vi "Node Type.vi"(8 "error in (no error)":errorcluster, 11 "JSON Tree In":variant) -> (0 "error out":errorcluster, 2 "Value":variant, 3 "JSON Tree Out":variant, 5 "JSON Compatible Type":T1=enum."Unknown", 7 "JSON Type":T2=enum."Unknown")   [LabVIEW 2014, in "i3-json.lvlib"]
doc: "Returns the JSON Type and Value of a given node in a JSON Tree. If possible, will also tell if there is a compatible LabVIEW datatype."
uses:
  i3-json.lvlib
  JSON Types/JSON Type.ctl
  JSON Types/JSON Compatible Type.ctl
  JSON Types/JSON Variant Attribute.ctl
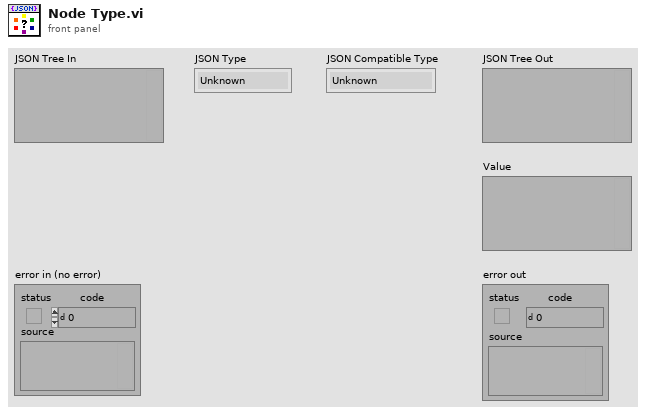
[diagram p1: front panel]
types:
  T1 = typedef "i3-json.lvlib/JSON Compatible Type.ctl" = enum16{"1D Double Array", "1D String Array", "1D Boolean Array", "Unknown"}
  T2 = typedef "i3-json.lvlib/JSON Type.ctl" = enum8{"JSON Compatible", "JSON Array", "JSON Object", "JSON Null", "Double", "String", "Boolean", "Unknown"}
  T3 = typedef "i3-json.lvlib/JSON Variant Attribute.ctl" = string
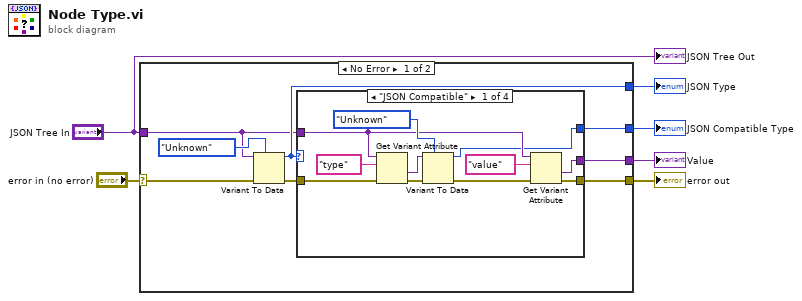
[diagram p0: block diagram]
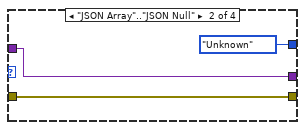
[diagram p2: hidden frame]
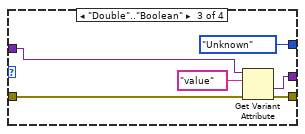
[diagram p3: hidden frame]
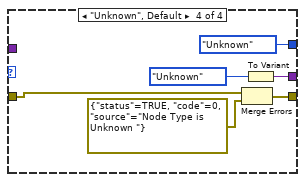
[diagram p4: hidden frame]
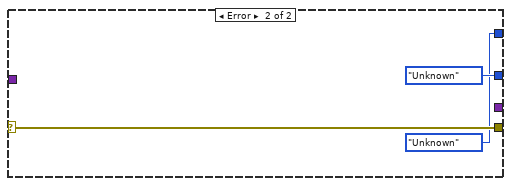
[diagram p5: hidden frame]
diagram:
  n1 = case shown="No Error" "error in (no error)" {
    selector: "error in (no error)" -> [w13 w43]
    tunnel: [w9 w43] -> w5
    tunnel: [w11 JSON_Compatible_Type."Unknown" ("JSON Compatible Type")] -> w4
    tunnel: [w10 JSON_Type."Unknown" ("JSON Type")] -> w3
    tunnel: "JSON Tree In" -> [w8 _]
    tunnel: [w7 _] -> w1
    frame No Error {
      n2 = Variant To Data(error in=w13, type=JSON_Type."Unknown" ("JSON Type"), Variant=w8) -> (data=w10:T2, error out=w12:errorcluster)
      n3 = case shown="\"JSON Compatible\"" w10 {
        tunnel: w8 -> [w17 w26 w33 _]
        tunnel: w12 -> [w25 w27 w31 w37]
        tunnel: [w15 JSON_Compatible_Type."Unknown" ("JSON Compatible Type") JSON_Compatible_Type."Unknown" ("JSON Compatible Type") JSON_Compatible_Type."Unknown" ("JSON Compatible Type")] -> w11
        tunnel: [w19 w27 w30 w35] -> w9
        tunnel: [w16 w26 w29 w40] -> w7
        frame "JSON Compatible" {
          n4 = Get Variant Attribute(Variant=w17, name=T3 "type" ("JSON Variant Attribute"), error in=w25) -> (value=w22:variant, error out=w23:errorcluster)  [unwired: 1 in, 2 out]
          n5 = Variant To Data(error in=w23, type=JSON_Compatible_Type."Unknown" ("JSON Compatible Type"), Variant=w22) -> (data=w15:T1, error out=w20:errorcluster)
          n6 = Get Variant Attribute(Variant=w17, name=T3 "value" ("JSON Variant Attribute"), error in=w20) -> (value=w16:variant, error out=w19:errorcluster)  [unwired: 1 in, 2 out]
        }
        frame "JSON Array".."JSON Null" {
        }
        frame "Double".."Boolean" {
          n7 = Get Variant Attribute(Variant=w33, name=T3 "value" ("JSON Variant Attribute"), error in=w31) -> (value=w29:variant, error out=w30:errorcluster)  [unwired: 1 in, 2 out]
        }
        frame "Unknown", Default {
          n8 = Merge Errors(w37, errorcluster {"status"=TRUE, "code"=0, "source"="Node Type is Unknown "} ("error out")) -> (w35:errorcluster)
          n9 = To Variant(anything=JSON_Type."Unknown" ("JSON Type")) -> (Variant=w40:variant)
        }
      }
    }
    frame Error {
    }
  }
  "error out" <- w5
  "JSON Compatible Type" <- w4
  "JSON Type" <- w3
  "Value" <- w1
  "JSON Tree Out" <- "JSON Tree In"
